vi "4Pi AA Delay X Frames.vi"(0 "Camera Notifier Name":string, 11 "Error In":errorcluster, 13 "Wait No. (1)":u32=1) -> (4 "Camera Notifier Name (Dup)":string, 15 "Error Out":errorcluster)   [LabVIEW 2016]
uses:
  Device Library/Cameras/Hamamatsu/Orca Flash/Orca Flash Controls/Orca Flash Actions.ctl
  Device Library/Cameras/Camera Controls/Camera IMAQ Key Info.ctl
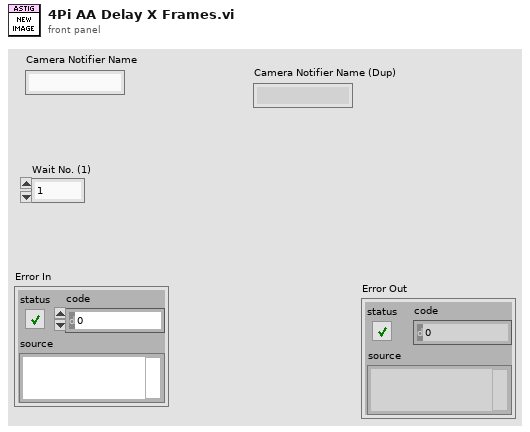
[diagram p1: front panel]
types:
  T1 = typedef "Camera IMAQ Key Info.ctl" = cluster{"Frame":u32, "Sensor Height":i32, "Sensor Width":i32, "ROI Height":i32, "ROI Width":i32, "ROI Enable?":bool, "Bit per Pixel":u8}
  T2 = typedef "Orca Flash Actions.ctl" = enum16{"IDLE", "PREVIEW", "RECORD", "Record Settings", "SETPARAM", "GETPARAM", "SETROI", "GETROI", "PROGRESSIVE MODE", "AREA MODE", "STATUS", "QUIT"}
  T3 = typedef "IMAQ Image.ctl" = refnum<image>
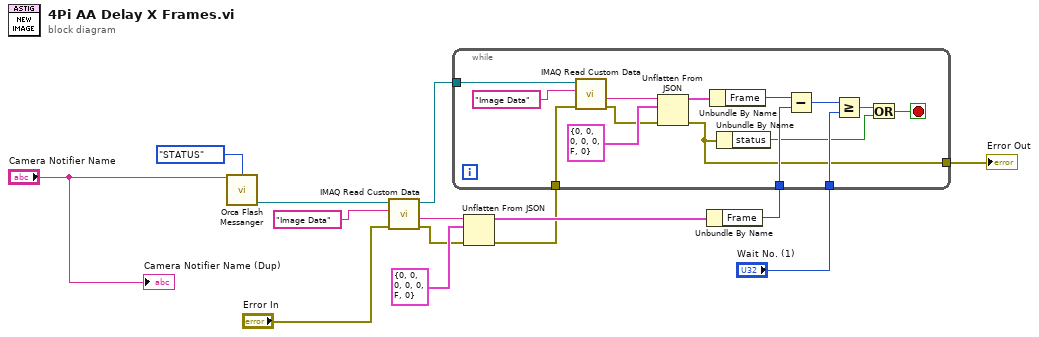
[diagram p0: block diagram]
diagram:
  n1 = call "Orca Flash Messanger.vi"("Notifier Name"="Camera Notifier Name", "Camera Actions"=Orca_Flash_Actions."STATUS") -> ("Image Ref"=w9:T3)  [unwired: 9 in, 4 out]
  n2 = call "IMAQ Read Custom Data"("error in (no error)"="Error In", "Key"="Image Data", "Image"=w9) -> ("error out"=w4:errorcluster, "Custom Data Out"=w11:string, "Image (duplicate)"=w8:T3)  [unwired: 6 in]
  n3 = Unflatten From JSON(JSON string=w11, type and defaults=T1 {"Frame"=0, "Sensor Height"=0, "Sensor Width"=0, "ROI Height"=0, "ROI Width"=0, "ROI Enable?"=FALSE, "Bit per Pixel"=0} ("Camera IMAQ Key Info"), error in (no error)=w4) -> (value=w13:T1, error out=w3:errorcluster)  [unwired: 4 in]
  n4 = Unbundle By Name(w13) -> ("Frame"=w7:u32)
  n5 = while {
    tunnel: w8 -> [w25]
    tunnel: w7 -> [w23]
    tunnel: "Wait No. (1)" -> [w21]
    tunnel: w3 -> [w20]
    tunnel: [w17] -> w1
    stop <- w15 stop-if-true
    n6 = call "IMAQ Read Custom Data"("error in (no error)"=w20, "Key"="Image Data", "Image"=w25) -> ("error out"=w19:errorcluster, "Custom Data Out"=w27:string)  [unwired: 6 in, 1 out]
    n7 = Unflatten From JSON(JSON string=w27, type and defaults=T1 {"Frame"=0, "Sensor Height"=0, "Sensor Width"=0, "ROI Height"=0, "ROI Width"=0, "ROI Enable?"=FALSE, "Bit per Pixel"=0} ("Camera IMAQ Key Info"), error in (no error)=w19) -> (value=w29:T1, error out=w17:errorcluster)  [unwired: 4 in]
    n8 = Unbundle By Name(w29) -> ("Frame"=w24:u32)
    n9 = Unbundle By Name(w17) -> ("status"=w16:bool)
    n10 = Subtract(x=w24, y=w23) -> (x-y=w22:u32)
    n11 = Greater Or Equal?(x=w22, y=w21) -> (x >= y?=w18:bool)
    n12 = Or(x=w18, y=w16) -> (x .or. y?=w15:bool)
  }
  "Error Out" <- w1
  "Camera Notifier Name (Dup)" <- "Camera Notifier Name"
